vi "Read Rig Config.vi"(8 "error in":errorcluster, 11 "path":path) -> (0 "error out":errorcluster, 2 "plugin class path":path, 3 "Rig Config":T1)   [LabVIEW 2026]
doc: "Reads a rig config JSON file and parses it into a Rig Config cluster; the plugin class path is the rig file folder joined with plugin_class. An empty path returns error 7; a missing file or JSON error is passed out; a rig with no channels returns error 5002. AF-free."
uses:
  Typedefs/Channel Definition.ctl
  Typedefs/Rig Config.ctl
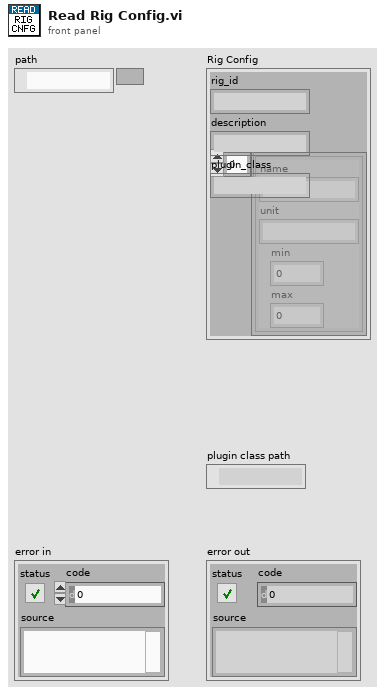
[diagram p1: front panel]
types:
  T1 = typedef "Rig Config.ctl" = cluster{"rig_id":string, "description":string, "plugin_class":string, "channels":T2[]}
  T2 = typedef "Channel Definition.ctl" = cluster{"name":string, "unit":string, "min":dbl, "max":dbl}
  T3 = cluster{"rig_id":string, "description":string, "plugin_class":string, "channels":cluster{"name":string, "unit":string, "min":dbl, "max":dbl}[]}
  T4 = cluster{"name":string, "unit":string, "min":dbl, "max":dbl}[]
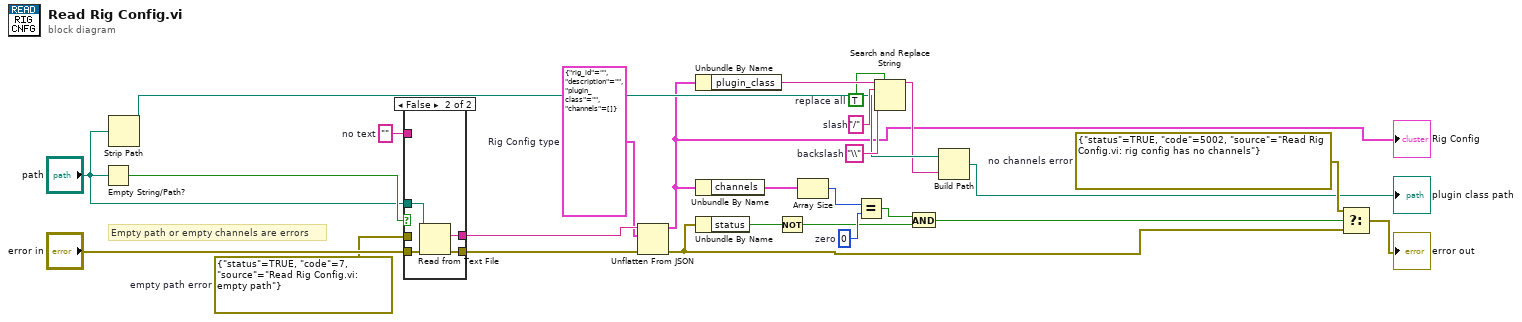
[diagram p0: block diagram]
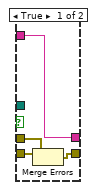
[diagram p2: hidden frame]
diagram:
  w6 = TRUE  # replace all
  w7 = "\\"  # backslash
  w8 = "/"  # slash
  w24 = ""  # no text
  w13 = errorcluster {"status"=TRUE, "code"=5002, "source"="Read Rig Config.vi: rig config has no channels"}  # no channels error
  w25 = errorcluster {"status"=TRUE, "code"=7, "source"="Read Rig Config.vi: empty path"}  # empty path error
  w16 = 0  # zero
  w21 = T3 {"rig_id"="", "description"="", "plugin_class"="", "channels"=[]}  # Rig Config type
  # "Empty path or empty channels are errors"
  n1 = Empty String/Path?(string/path="path") -> (empty?=w23:bool)
  n2 = Strip Path(path="path") -> (stripped path=w5:path)  [unwired: 1 out]
  n3 = case shown="False" w23 {
    tunnel: "path" -> [_ w34]
    tunnel: "error in" -> [w30 w33]
    tunnel: w25 -> [w29 _]
    tunnel: [w28 w32] -> w22
    tunnel: w24 -> [w28 _]
    tunnel: [w27 w31] -> w20
    frame True {
      n4 = Merge Errors(w30, w29) -> (w27:errorcluster)
    }
    frame False {
      n5 = Read from Text File(file (use dialog)=w34, error in=w33) -> (text=w32:string, error out=w31:errorcluster)  [unwired: 2 in, 2 out]
    }
  }
  n6 = Unflatten From JSON(JSON string=w22, type and defaults=w21, error in (no error)=w20) -> (value=w3:T3, error out=w11:errorcluster)  [unwired: 4 in]
  "Rig Config" <- w3
  n7 = Unbundle By Name(w3) -> ("plugin_class"=w9:string)
  n8 = Unbundle By Name(w3) -> ("channels"=w19:T4)
  n9 = Unbundle By Name(w11) -> ("status"=w18:bool)
  n10 = Not(x=w18) -> (.not. x?=w14:bool)
  n11 = Array Size(array=w19) -> (size(s)=w17:i32)
  n12 = Equal?(x=w17, y=w16) -> (x = y?=w15:bool)
  n13 = Search and Replace String(replace all?=w6, input string=w9, search string=w8, replace string=w7) -> (result string=w4:string)  [unwired: 4 in, 3 out]
  n14 = And(x=w15, y=w14) -> (x .and. y?=w12:bool)
  n15 = Build Path(base path=w5, name or relative path=w4) -> (appended path=→"plugin class path":path)
  n16 = Select(t=w13, s=w12, f=w11) -> (s? t:f=→"error out":errorcluster)
